vi "LV to ITX XY AutoPlot.vi"(4 "X,Y Log":i32[](array[numeric]), 6 "X,Y Labels":string[](array[string])=["x label", "y label"], 7 "Notes":string, 8 "error in":errorcluster, 10 "XY-Data []":cluster{"X  array":dbl[], "Y  Array":dbl[]}[](array[cluster]), 11 "path":path=path "C:/Users/voodoo.SEAGATE/Desktop/datatest") -> (0 "error out":errorcluster, 3 "file":path=path "C:/Users/voodoo.SEAGATE/Desktop/datatest/datatest.000019.itx")   [LabVIEW 2019, in "LV-Data.ITX.lvclass"]
doc: "Write your XY data to ITX file. This AutoPlot VI adds commands to automatically create a graph in Igor to quickly view your data.\n\n-- path: base path to save data\n-- filename: base filename\n-- Notes: add any notes here to help you remember what experiment you did\n-- XY Array: Array of Clusters (ie, Array of XY graphs)\n-- wavenames: Give each data array a unique name such as \"time, bias, current,...\"\n-- X,Y Labels: For plotting in Igor. Can be ignored.\n-- X,Y Log: Do you wan to show X or Y on Log scale in Igor?"
uses:
  LV-Data.ITX.lvclass
  LV-Data/Typedefs/Operation--enum.ctl
  LV-Data/Typedefs/File Type--enum.ctl
  LV-Data/LV-Data.lvclass/LV-Data.ctl
  LV-Data.ITX.lvclass/LV-Data.ITX.ctl
  4e7104cf-761e-49f4-a8a0-3f14be840846.vi
  4e7104cf-761e-49f4-a8a0-3f14be840846.vi/6646e538-63a8-4ded-86ed-1776b35804e5.vi
  <vilib>/AdvancedString/1D String Array to Delimited String.vi
  private/Variant to ITX Wave.vi
  private/Commands to ITX.vi
  private/Notes to ITX.vi
  LV-Data/LV-Data.lvclass
  ITX Commands/ITX Commands.lvclass
panel:
  # "Below are relevant for creating graphs in Igor"
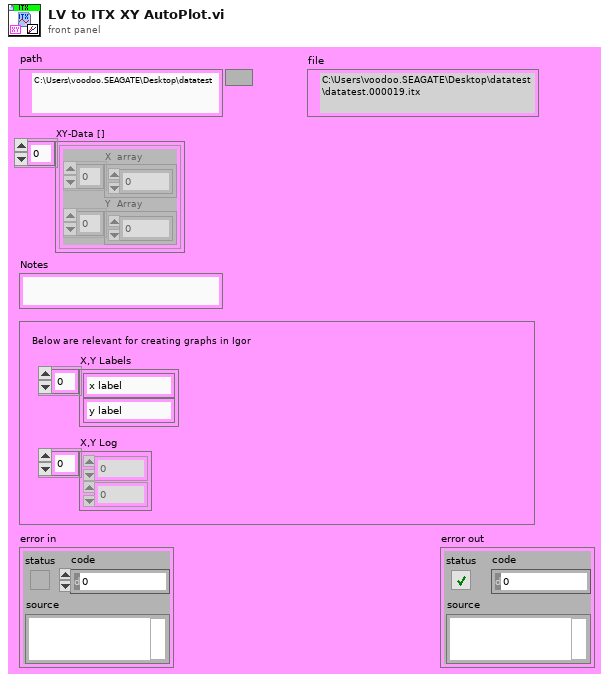
[diagram p1: front panel]
types:
  T1 = typedef "LV-Data.lvclass/File Type--enum.ctl" = enum16{"DAT", "ITX", "TDMS", "VI"}
  T2 = typedef "LV-Data.lvclass/Operation--enum.ctl" = enum16{"Read", "Write", "Write + Append"}
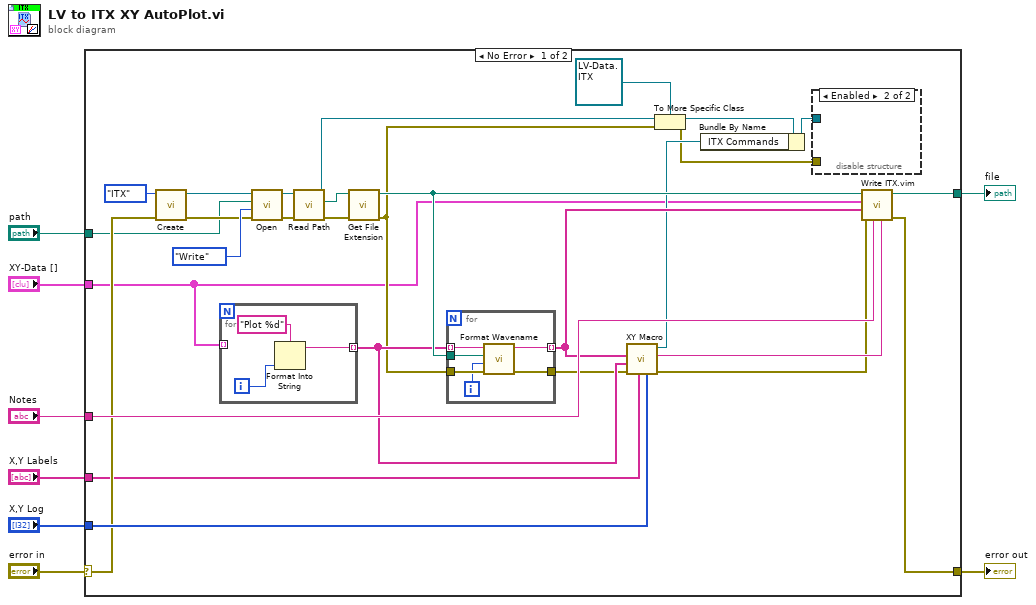
[diagram p0: block diagram]
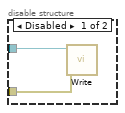
[diagram p2: hidden frame]
diagram:
  n1 = case shown="No Error" "error in" {
    selector: "error in" -> [w24 w50]
    tunnel: "path" -> [w22 w49]
    tunnel: "X,Y Labels" -> [w19 _]
    tunnel: [w37 w49] -> w6
    tunnel: "X,Y Log" -> [w36 _]
    tunnel: "XY-Data []" -> [w9 _]
    tunnel: [w35 w50] -> w2
    tunnel: "Notes" -> [w33 _]
    frame No Error {
      n2 = call "Create.vi"("error in (no error)"=w24, "File Type"=File_Type--enum."ITX") -> ("error out"=w23:errorcluster, "Data out"=w25:refnum<class "LV-Data.lvclass">)  [unwired: 8 in]
      n3 = for {
        tunnel: w9 -> [_] mode=indexing
        tunnel: [w38] -> w20 mode=indexing
        i -> [w40]
        n4 = Format Into String(format string="Plot %d", w40) -> (resulting string=w38:string)  [unwired: 2 in, 1 out]
      }
      n5 = call-dynamic "Open.vi"("error in (no error)"=w23, "Operation"=Operation--enum."Write", "Path"=w22, "Data in"=w25) -> ("error out"=w28:errorcluster, "Data out"=w29:refnum<class "LV-Data.lvclass">)  [unwired: 6 in]
      n6 = call "Read Path.vi"("error in (no error)"=w28, "Data Save"=w29) -> ("error out"=w31:errorcluster, "Path"=w32:path, "Data Save out"=w16:refnum<class "LV-Data.lvclass">)  [unwired: 7 in]
      n7 = call <vilib>:"Get File Extension.vi"("error in (no error)"=w31, "file"=w32) -> ("error out"=w11:errorcluster, "dup file"=w30:path)  [unwired: 5 in, 3 out]
      n8 = for {
        tunnel: w20 -> [w46] mode=indexing
        tunnel: [w43] -> w21 mode=indexing
        tunnel: w30 -> [w41]
        tunnel: w11 -> [w45]
        tunnel: [w44] -> w18
        i -> [w42]
        n9 = call "Format Wavename.vi"("error in (no error)"=w45, "Index"=w42, "Path"=w41, "Name"=w46) -> ("error out"=w44:errorcluster, "Formatted wavename"=w43:string)  [unwired: 6 in]
      }
      n10 = call "XY Macro.vi"("X,Y Log"=w36, "X,Y Labels"=w19, "error in (no error)"=w18, "Plot labels"=w20, "wavenames"=w21) -> ("error out"=w17:errorcluster, "Commands"=w34:string, "ITX Commands out"=w14:refnum<class "ITX Commands.lvclass">)  [unwired: 4 in]
      n11 = To More Specific Class(target class=refnum<class "LV-Data.ITX.lvclass"> refnum ("LV-Data.ITX.lvclass"), reference=w16, error in=w11) -> (specific class reference=w13:refnum<class "LV-Data.ITX.lvclass">, error out=w10:errorcluster)
      n12 = Bundle By Name(cluster=w13, "ITX Commands"=w14) -> (w12:refnum<class "LV-Data.ITX.lvclass">)
      n13 = disable-structure shown="Enabled" {
        disable-tunnel: w12 -> [w48 _]
        disable-tunnel: w10 -> [w47 _]
        frame Disabled {
          n14 = call-dynamic "Write.vi"("error in (no error)"=w47, "Data.ITX in"=w48) -> ()  [unwired: 7 in, 3 out]
        }
        frame Enabled {
        }
      }
      n15 = call "Write ITX.vim"("commands"=w34, "notes"=w33, "error in"=w17, "wavename"=w21, "values"=w9, "filename"=w30) -> ("error out"=w35:errorcluster, "filename out"=w37:path)  [unwired: 3 in, 1 out]
    }
    frame Error {
    }
  }
  "file" <- w6
  "error out" <- w2
